vi "Check I2C Device.vi"(8 "error in (no error)":errorcluster) -> (0 "error out":errorcluster)   [LabVIEW 2020, in "wiringPi.lvlib"]
doc: "<b>_______________________________________________________________</b>\n** Author: Juan José Villacorta\n** LabVIEW wrapper for C library <b> wiringPi </b>,\n** https://github.com/WiringPi/WiringPi\n<b>_______________________________________________________________</b>\n/*\n * Check if the SPI device is present\n**********************************************************************************\n*/"
uses:
  wiringPi.lvlib
  <vilib>/ErrorRing/Error Ring.xnode
  <vilib>/Utility/error.llb/Error Cluster From Error Code.vi
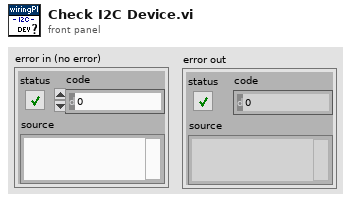
[diagram p1: front panel]
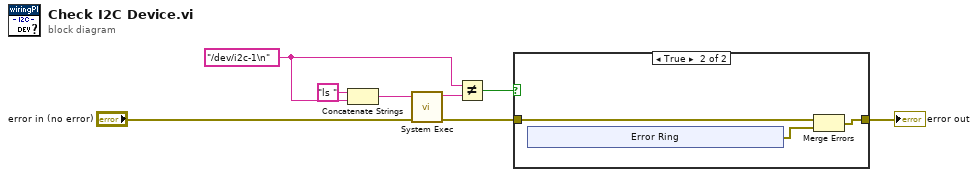
[diagram p0: block diagram]
diagram:
  w1 = "/dev/i2c-1\n" ("format string")
  n1 = Concatenate Strings("ls " ("string"), w1) -> (w7:string)
  n2 = call <vilib>:"System Exec.vi"("error in (no error)"="error in (no error)", "command line"=w7) -> ("error out"=w3:errorcluster, "standard output"=w5:string)  [unwired: 6 in, 2 out]
  n3 = Not Equal?(x=w1, y=w5) -> (x != y?=w4:bool)
  n4 = case shown="True" w4 {
    tunnel: w3 -> [w9 w11]
    tunnel: [w9 w10] -> w2
    frame False {
    }
    frame True {
      n5 = xnode "Error Ring"() -> ("error out"=w12:errorcluster)
      n6 = Merge Errors(w11, w12) -> (w10:errorcluster)
    }
  }
  "error out" <- w2
